vi "Relative2Absolute.vi"(0 "机器人语音指令数据簇":T1, 1 "now_pose_X":dbl, 2 "now_pose_Y":dbl, 3 "now_pose_Rot_deg":dbl) -> (7 "x":dbl, 8 "y":dbl, 10 "Rot_deg":dbl)   [LabVIEW 2014]
uses:
  <vilib>/imath/engines/lvmath2/RunTimeEngine/NodeEndStatement/NIMS_NodeEndStatement_Output.vi
  <instcachedir>/0/NIMS_NodeEndStatement_Output_53EC0D466D134D7ABD903AC30B43404B.lvgen/NIMS_NodeEndStatement_Output_53EC0D466D134D7ABD903AC30B43404B_001.vi
  <vilib>/imath/engines/lvmath2/RunTimeEngine/ErrorHandling/NIMS_Finalize Error.vi
panel:
  out "f":dbl
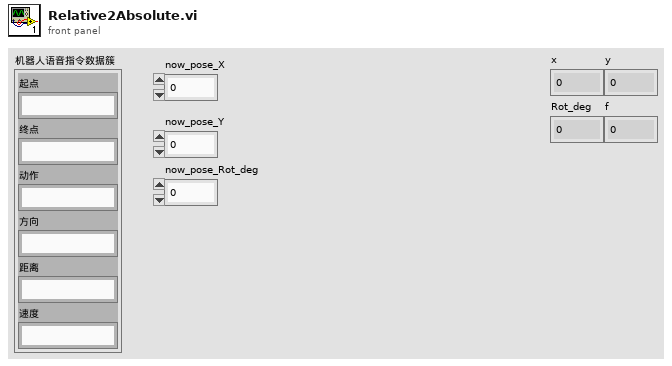
[diagram p1: front panel]
types:
  T1 = cluster{"起点":string, "终点":string, "动作":string, "方向":string, "距离":string, "速度":string}
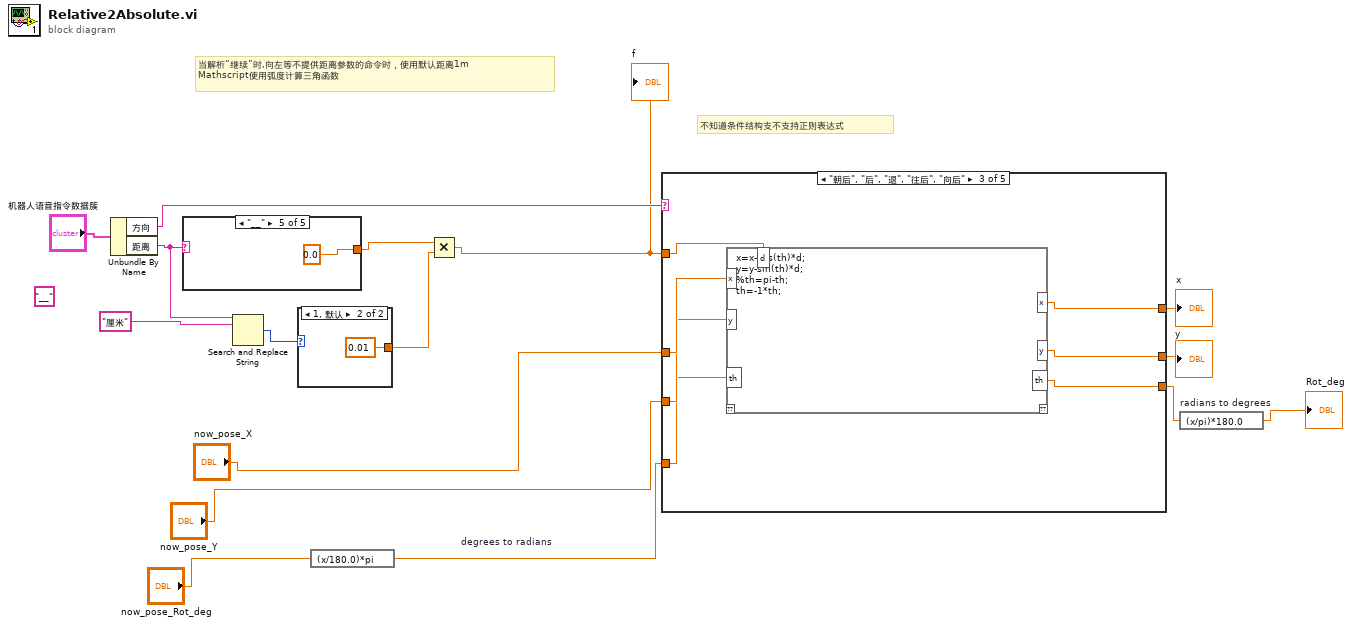
[diagram p0: block diagram]
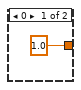
[diagram p2: hidden frame]
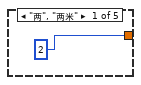
[diagram p3: hidden frame]
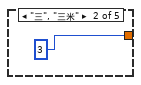
[diagram p4: hidden frame]
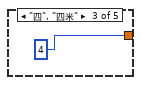
[diagram p5: hidden frame]
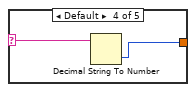
[diagram p6: hidden frame]
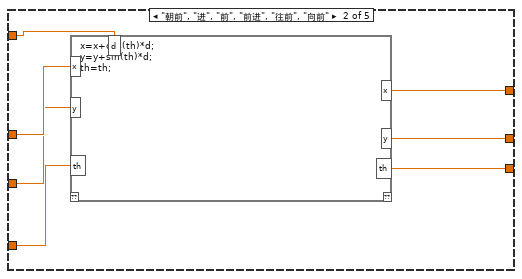
[diagram p8: hidden frame]
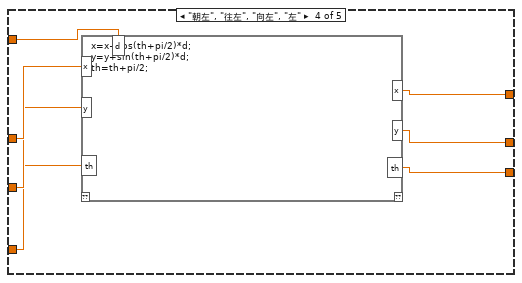
[diagram p9: hidden frame]
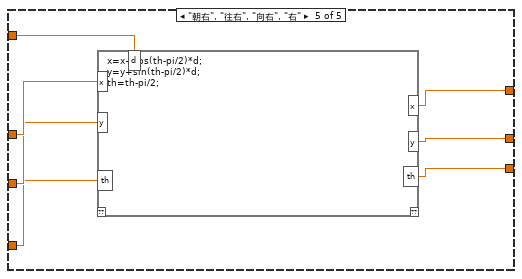
[diagram p10: hidden frame]
diagram:
  (unwired) "__" ("y")
  # "不知道条件结构支不支持正则表达式"
  # "当解析“继续”时,向左等不提供距离参数的命令时，使用默认距离1m\nMathscript使用弧度计算三角函数"
  n1 = Unbundle By Name("机器人语音指令数据簇") -> ("方向"=w15:string, "距离"=w8:string)
  n2 = case shown="\"__\"" w8 {
    selector: w8 -> [_ _ _ w21 _]
    tunnel: [2 ("f") 3 ("f") 4 ("f") w20 0.0] -> w9
    frame "两", "两米" {
    }
    frame "三", "三米" {
    }
    frame "四", "四米" {
    }
    frame Default {
      n3 = Decimal String To Number(string=w21) -> (number=w20:i32)  [unwired: 2 in, 1 out]
    }
    frame "__" {
    }
  }
  n4 = Search and Replace String(input string=w8, search string="厘米" ("搜索字符串")) -> (number of replacements=w6:i32)  [unwired: 6 in, 3 out]
  n5 = case shown="1, 默认" w6 {
    tunnel: [1.0 ("y") 0.01 ("y")] -> w5
    frame 0 {
    }
    frame 1, Default {
    }
  }
  n6 = expression code="(x/180.0)*pi" "degrees to radians"("now_pose_Rot_deg") -> (w14:dbl)
  n7 = Multiply(x=w9, y=w5) -> (x*y=w4:dbl)
  "f" <- w4
  n8 = case shown="\"朝后\", \"后\", \"退\", \"往后\", \"向后\"" w15 {
    tunnel: "now_pose_X" -> [w27 w34 w85 w139 w203]
    tunnel: "now_pose_Y" -> [w26 w33 w84 w138 w202]
    tunnel: w14 -> [w25 w32 w83 w137 w201]
    tunnel: w4 -> [_ w28 w86 w140 w204]
    tunnel: [w27 w31 w82 w136 w200] -> w13
    tunnel: [w26 w30 w81 w135 w199] -> w12
    tunnel: [w25 w29 w80 w134 w198] -> w11
    frame "_", Default {
    }
    frame "朝前", "进", "前", "前进", "往前", "向前" {
      n9 = mathscript code="x=x+cos(th)*d;\ny=y+sin(th)*d;\nth=th;"("x"=w34, "y"=w33, "th"=w32, "d"=w28) -> ("x"=w31:dbl, "y"=w30:dbl, "th"=w29:dbl)  [unwired: 1 in, 1 out]
    }
    frame "朝后", "后", "退", "往后", "向后" {
      n10 = mathscript code="x=x-cos(th)*d;\ny=y-sin(th)*d;\n%th=pi-th;\nth=-1*th;"("x"=w85, "y"=w84, "th"=w83, "d"=w86) -> ("x"=w82:dbl, "y"=w81:dbl, "th"=w80:dbl)  [unwired: 1 in, 1 out]
    }
    frame "朝左", "往左", "向左", "左" {
      n11 = mathscript code="x=x+cos(th+pi/2)*d;\ny=y+sin(th+pi/2)*d;\nth=th+pi/2;"("x"=w139, "y"=w138, "th"=w137, "d"=w140) -> ("x"=w136:dbl, "y"=w135:dbl, "th"=w134:dbl)  [unwired: 1 in, 1 out]
    }
    frame "朝右", "往右", "向右", "右" {
      n12 = mathscript code="x=x+cos(th-pi/2)*d;\ny=y+sin(th-pi/2)*d;\nth=th-pi/2;"("x"=w203, "y"=w202, "th"=w201, "d"=w204) -> ("x"=w200:dbl, "y"=w199:dbl, "th"=w198:dbl)  [unwired: 1 in, 1 out]
    }
  }
  "x" <- w13
  "y" <- w12
  n13 = expression code="(x/pi)*180.0" "radians to degrees"(w11) -> (→"Rot_deg":dbl)
